vi "VIH Dialog - Project File List - Shortcut Menu Handler.vi"(6 "Menu Tag":string, 7 "Options":cluster{"Called from Master":bool}, 8 "Files":cluster{"Type":T1, "Path":path}[](array[cluster]), 10 "MenuRef":refnum<k9>, 11 "Event Type":T2) -> (3 "States spec":string)   [LabVIEW 2014]
doc: "::: VI Helpeks :::\nCopyright (c) 2000-2026 Konstantin Shifershteyn. All rights reserved."
uses:
  <vilib>/event_ctls.llb/lveventtype.ctl
  _VIH HelpGen - Palette.llb/VIH HelpGen Typedef - Palette - Item Type Enum.ctl
  _VIH Support Library.llb/VIH Utility - MENU - Create Menu (String).vi
panel:
  # "VI Helpeks\nCopyright (c) 2012-2026 Konstantin Shifershteyn"
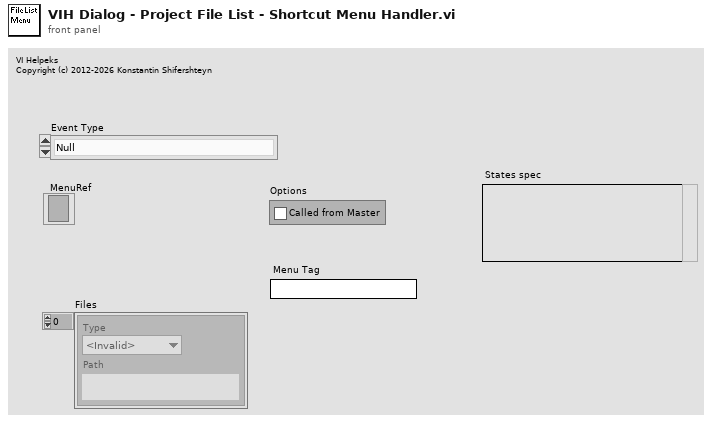
[diagram p1: front panel]
types:
  T1 = typedef "VIH HelpGen Typedef - Palette - Item Type Enum.ctl" = enum32{"<Invalid>", "<unknown>", "VI", "Menu", "LV Func", "Express VI", "Poly VI", "CTL", "HTML"}
  T2 = typedef "lveventtype.ctl" = enum32{"Null", "Timeout", "Annotation Menu Selection", "Annotation Menu Selection?", "App Instance Close", "App Instance Close?", "Autoscale Range Change", "Bookmark Info Change", "Cell Edit", "Cell Edit?", "Cursor Grab", "Cursor Grab?", "Cursor Menu Selection", "Cursor Menu Selection?", "Cursor Move", "Cursor Release", "Data Change", "Direction Change", "Display State Change", "Drag Ended", "Drag Enter", "Drag Leave", "Drag Over", "Drag Source Update", "Drag Starting", "Drag Starting?", "Drop", "Exec State Change", "Key Down", "Key Down?", "Key Repeat", "Key Repeat?", "Key Up", "Listbox Double Click", "Menu Activation?", "Menu Selection (App)", "Menu Selection? (App)", "Menu Selection (User)", "Mouse Down", "Mouse Down?", "Mouse Enter", "Mouse Leave", "Mouse Move", "Mouse Up", "Mouse Wheel", "NI Security User Change (App)", "Pane Size", "Panel Close", "Panel Close?", "Panel Resize", "Plot Attribute Change", "Scale Range Change", "Shortcut Menu Activation?", "Shortcut Menu Selection (App)", "Shortcut Menu Selection? (App)", "Shortcut Menu Selection (User)", "Tree Double Click", "Tree Drag", "Tree Drag?", "Tree Drop", "Tree Drop?", "Tree Item Close", "Tree Item Close?", "Tree Item Open", "Tree Item Open?", "User Event", "Value Change"}
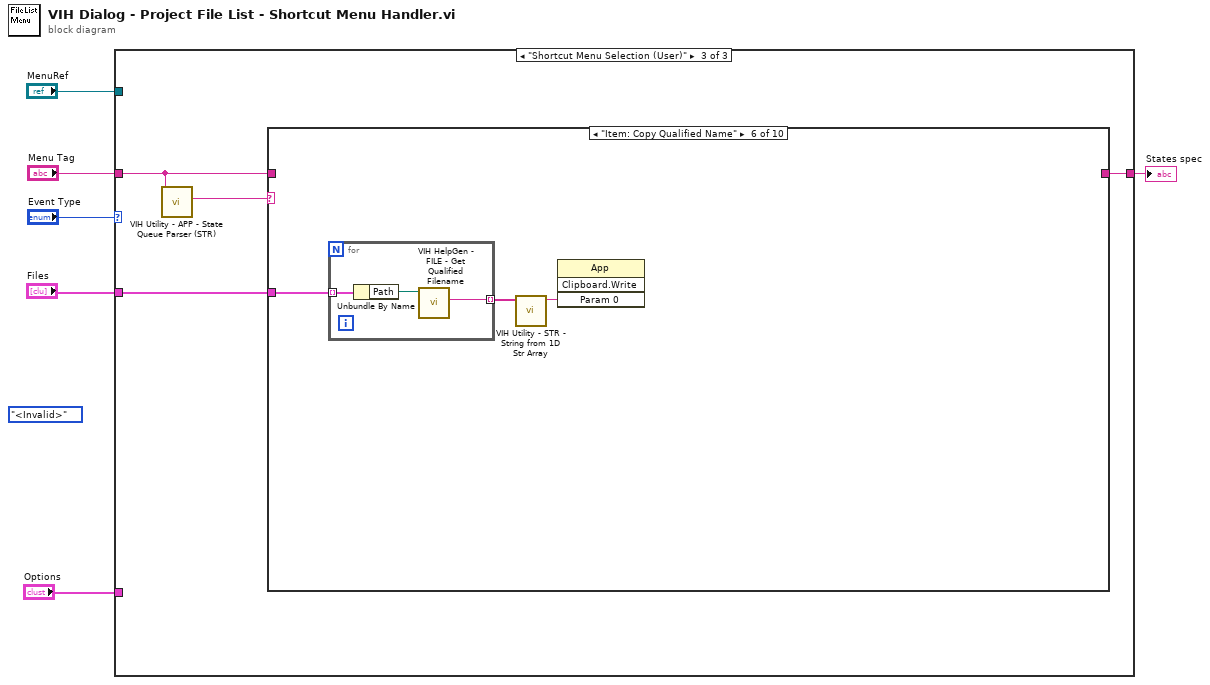
[diagram p0: block diagram]
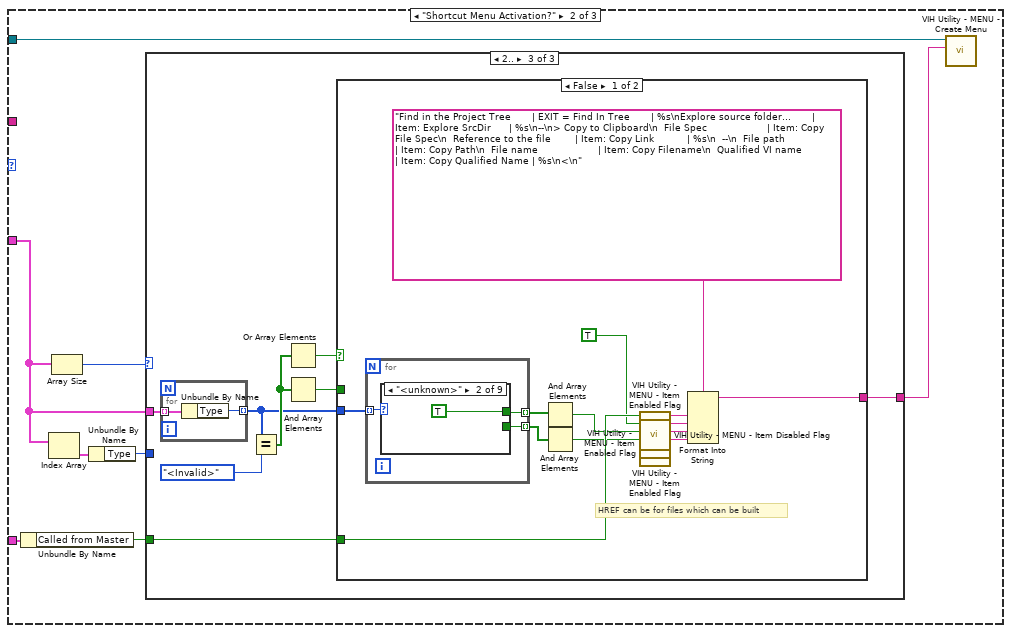
[diagram p3: hidden frame]
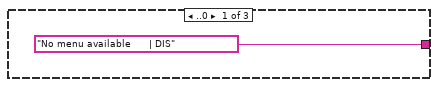
[diagram p4: hidden frame]
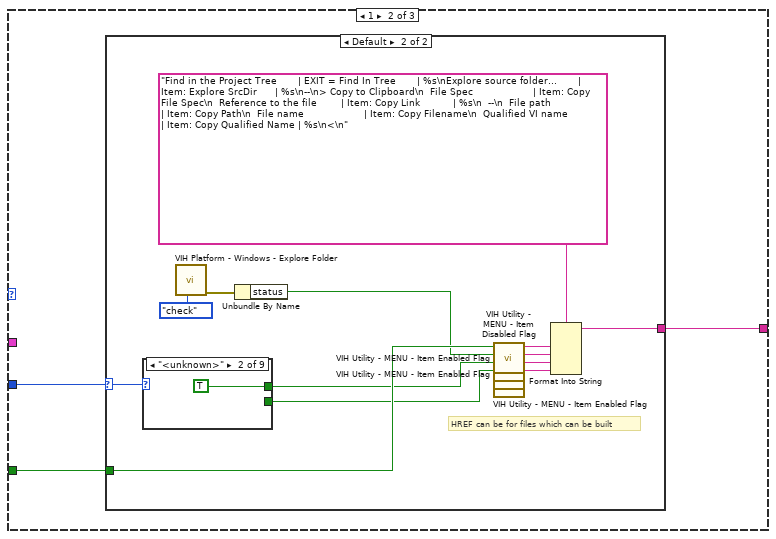
[diagram p5: hidden frame]
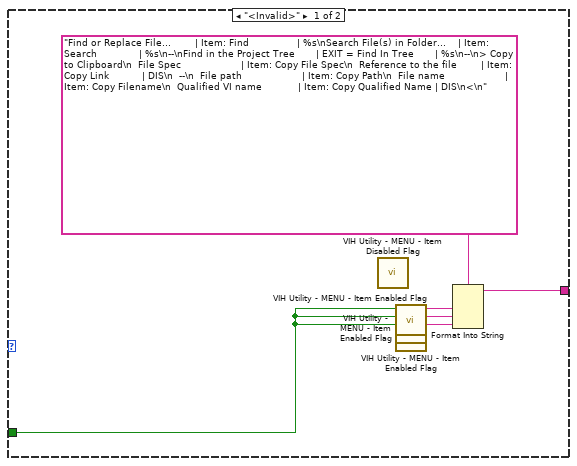
[diagram p6: hidden frame]
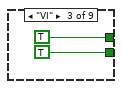
[diagram p8: hidden frame]
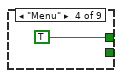
[diagram p9: hidden frame]
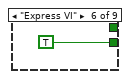
[diagram p11: hidden frame]
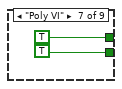
[diagram p12: hidden frame]
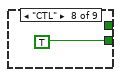
[diagram p13: hidden frame]
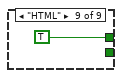
[diagram p14: hidden frame]
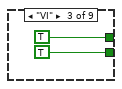
[diagram p16: hidden frame]
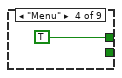
[diagram p17: hidden frame]
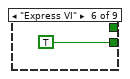
[diagram p19: hidden frame]
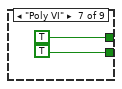
[diagram p20: hidden frame]
diagram:
  (unwired) VIH_HelpGen_Typedef_-_Palette_-_Item_Type_Enum."<Invalid>" ("Type")
  n1 = case shown="\"Shortcut Menu Selection (User)\"" "Event Type" {
    tunnel: "MenuRef" -> [_ w14 _]
    tunnel: [_ _ w92] -> w4
    tunnel: "Menu Tag" -> [_ _ w93]
    tunnel: "Files" -> [_ w7 w91]
    tunnel: "Options" -> [_ w12 _]
    frame Default {
    }
    frame "Shortcut Menu Activation?" {
      n2 = Unbundle By Name(w12) -> ("Called from Master"=w11:bool)
      n3 = Index Array(array=w7) -> (element=w9:cluster{"Type":T1, "Path":path})  [unwired: 1 in]
      n4 = Array Size(array=w7) -> (size(s)=w10:i32)
      n5 = Unbundle By Name(w9) -> ("Type"=w8:T1)
      n6 = case shown="2.." w10 {
        tunnel: ["No menu available      | DIS" w18 w54] -> w13
        tunnel: w11 -> [_ w17 w53]
        tunnel: w8 -> [_ w16 _]
        tunnel: w7 -> [_ _ w52]
        frame ..0 {
        }
        frame 1 {
          n7 = case shown="Default" w16 {
            selector: w16 -> [_ w33]
            tunnel: [w23 w36] -> w18
            tunnel: w17 -> [w19 w34]
            frame "<Invalid>" {
              n8 = call "VIH Utility - MENU - Item Disabled Flag.vi"() -> ()  [unwired: 11 in, 1 out]
              n9 = call "VIH Utility - MENU - Item Enabled Flag.vi"("Enable?"=w19) -> ("Disable flag"=w22:string)  [unwired: 10 in]
              n10 = call "VIH Utility - MENU - Item Enabled Flag.vi"("Enable?"=w19) -> ("Disable flag"=w21:string)  [unwired: 10 in]
              n11 = call "VIH Utility - MENU - Item Enabled Flag.vi"("Enable?"=w19) -> ("Disable flag"=w20:string)  [unwired: 10 in]
              n12 = Format Into String(format string="Find or Replace File...        | Item: Find                | %s\nSearch File(s) in Folder...    | Item: Search              | %s\n--\nFind in the Project Tree       | EXIT = Find In Tree       | %s\n--\n> Copy to Clipboard\n  File Spec                    | Item: Copy File Spec\n  Reference to the file        | Item: Copy Link           | DIS\n  --\n  File path                    | Item: Copy Path\n  File name                    | Item: Copy Filename\n  Qualified VI name            | Item: Copy Qualified Name | DIS\n<\n", w22, w21, w20) -> (resulting string=w23:string)  [unwired: 2 in, 1 out]
            }
            frame Default {
              # "HREF can be for files which can be built"
              n13 = case shown="\"<unknown>\"" w33 {
                tunnel: [_ TRUE TRUE TRUE _ _ TRUE _ TRUE] -> w27
                tunnel: [_ _ TRUE _ _ TRUE TRUE TRUE _] -> w26
                frame "<Invalid>" {
                }
                frame "<unknown>" {
                }
                frame "VI" {
                }
                frame "Menu" {
                }
                frame "LV Func" {
                }
                frame "Express VI" {
                }
                frame "Poly VI" {
                }
                frame "CTL" {
                }
                frame "HTML" {
                }
              }
              n14 = call "VIH Platform - Windows - Explore Folder.vi"("cmd (run)"=enum16{"run", "check"}."check") -> ("error out"=w30:errorcluster)  [unwired: 10 in]
              n15 = Unbundle By Name(w30) -> ("status"=w28:bool)
              n16 = call "VIH Utility - MENU - Item Enabled Flag.vi"("Enable?"=w34) -> ("Disable flag"=w35:string)  [unwired: 10 in]
              n17 = call "VIH Utility - MENU - Item Disabled Flag.vi"("Disable?"=w28) -> ("Disable flag"=w29:string)  [unwired: 10 in]
              n18 = call "VIH Utility - MENU - Item Enabled Flag.vi"("Enable?"=w27) -> ("Disable flag"=w32:string)  [unwired: 10 in]
              n19 = call "VIH Utility - MENU - Item Enabled Flag.vi"("Enable?"=w26) -> ("Disable flag"=w25:string)  [unwired: 10 in]
              n20 = Format Into String(format string="Find in the Project Tree       | EXIT = Find In Tree       | %s\nExplore source folder...       | Item: Explore SrcDir      | %s\n--\n> Copy to Clipboard\n  File Spec                    | Item: Copy File Spec\n  Reference to the file        | Item: Copy Link           | %s\n  --\n  File path                    | Item: Copy Path\n  File name                    | Item: Copy Filename\n  Qualified VI name            | Item: Copy Qualified Name | %s\n<\n", w35, w29, w32, w25) -> (resulting string=w36:string)  [unwired: 2 in, 1 out]
            }
          }
        }
        frame 2.. {
          n21 = for {
            tunnel: w52 -> [w90] mode=indexing
            tunnel: [w89] -> w47 mode=indexing
            n22 = Unbundle By Name(w90) -> ("Type"=w89:T1)
          }
          n23 = Equal?(x=w47, y=VIH_HelpGen_Typedef_-_Palette_-_Item_Type_Enum."<Invalid>" ("Type")) -> (x = y?=w50:bool[])
          n24 = Or Array Elements(Boolean array=w50) -> (logical OR=w49:bool)
          n25 = And Array Elements(Boolean array=w50) -> (logical AND=w48:bool)
          n26 = case shown="False" w49 {
            tunnel: [w66 w87] -> w54
            tunnel: w53 -> [w64 w81]
            tunnel: w48 -> [_ w80]
            tunnel: w47 -> [w60 _]
            frame False {
              # "HREF can be for files which can be built"
              n27 = for {
                tunnel: [w69] -> w62 mode=indexing
                tunnel: w60 -> [w70] mode=indexing
                tunnel: [w68] -> w57 mode=indexing
                n28 = case shown="\"<unknown>\"" w70 {
                  tunnel: [_ TRUE TRUE TRUE _ _ TRUE _ TRUE] -> w69
                  tunnel: [_ _ TRUE _ _ TRUE TRUE TRUE _] -> w68
                  frame "<Invalid>" {
                  }
                  frame "<unknown>" {
                  }
                  frame "VI" {
                  }
                  frame "Menu" {
                  }
                  frame "LV Func" {
                  }
                  frame "Express VI" {
                  }
                  frame "Poly VI" {
                  }
                  frame "CTL" {
                  }
                  frame "HTML" {
                  }
                }
              }
              n29 = And Array Elements(Boolean array=w62) -> (logical AND=w61:bool)
              n30 = And Array Elements(Boolean array=w57) -> (logical AND=w56:bool)
              n31 = call "VIH Utility - MENU - Item Enabled Flag.vi"("Enable?"=w64) -> ("Disable flag"=w65:string)  [unwired: 10 in]
              n32 = call "VIH Utility - MENU - Item Disabled Flag.vi"("Disable?"=TRUE) -> ("Disable flag"=w59:string)  [unwired: 10 in]
              n33 = call "VIH Utility - MENU - Item Enabled Flag.vi"("Enable?"=w61) -> ("Disable flag"=w63:string)  [unwired: 10 in]
              n34 = call "VIH Utility - MENU - Item Enabled Flag.vi"("Enable?"=w56) -> ("Disable flag"=w55:string)  [unwired: 10 in]
              n35 = Format Into String(format string="Find in the Project Tree       | EXIT = Find In Tree       | %s\nExplore source folder...       | Item: Explore SrcDir      | %s\n--\n> Copy to Clipboard\n  File Spec                    | Item: Copy File Spec\n  Reference to the file        | Item: Copy Link           | %s\n  --\n  File path                    | Item: Copy Path\n  File name                    | Item: Copy Filename\n  Qualified VI name            | Item: Copy Qualified Name | %s\n<\n", w65, w59, w63, w55) -> (resulting string=w66:string)  [unwired: 2 in, 1 out]
            }
            frame True {
              n36 = And(x=w80, y=w81) -> (x .and. y?=w82:bool)
              n37 = call "VIH Utility - MENU - Item Disabled Flag.vi"() -> ()  [unwired: 11 in, 1 out]
              n38 = call "VIH Utility - MENU - Item Enabled Flag.vi"("Enable?"=FALSE) -> ("Disable flag"=w84:string)  [unwired: 10 in]
              n39 = call "VIH Utility - MENU - Item Enabled Flag.vi"("Enable?"=w82) -> ("Disable flag"=w85:string)  [unwired: 10 in]
              n40 = call "VIH Utility - MENU - Item Enabled Flag.vi"("Enable?"=w81) -> ("Disable flag"=w88:string)  [unwired: 10 in]
              n41 = Format Into String(format string="Find or Replace File...        | Item: Find                | %s\nSearch File(s) in Folder...    | Item: Search              | %s\n--\nFind in the Project Tree       | EXIT = Find In Tree       | %s\n--\n> Copy to Clipboard\n  File Spec                    | Item: Copy File Spec\n  Reference to the file        | Item: Copy Link           | DIS\n  --\n  File path                    | Item: Copy Path\n  File name                    | Item: Copy Filename\n  Qualified VI name            | Item: Copy Qualified Name | DIS\n<\n", w84, w85, w88) -> (resulting string=w87:string)  [unwired: 2 in, 1 out]
            }
          }
        }
      }
      n42 = call-poly "VIH Utility - MENU - Create Menu.vi"("Menu Description"=w13, "menu"=w14) -> ()  [unwired: 8 in, 2 out]
    }
    frame "Shortcut Menu Selection (User)" {
      n43 = call "VIH Utility - APP - State Queue Parser (STR).vi"("input queue"=w93) -> ("state"=w94:string)  [unwired: 5 in, 3 out]
      n44 = case shown="\"Item: Copy Qualified Name\"" w94 {
        tunnel: [w95 _ _ _ _ _ _ w133 w142 _] -> w92
        tunnel: w93 -> [w96 _ _ _ _ _ _ _ _ _]
        tunnel: w91 -> [_ w103 w109 w116 w121 w127 _ w137 w141 w151]
        frame Default {
          n45 = Match Pattern(string=w96, regular expression=";$") -> (offset past match=w97:i32)  [unwired: 1 in, 3 out]
          n46 = case shown="..-1" w97 {
            tunnel: w96 -> [w101 w102]
            tunnel: [w100 w102] -> w95
            frame ..-1 {
              n47 = Concatenate Strings(w101, ";" ("string")) -> (w100:string)
            }
            frame 0.. {
            }
          }
        }
        frame "Item: Copy File Spec" {
          n48 = for {
            tunnel: [w108] -> w105 mode=indexing
            tunnel: w103 -> [w107] mode=indexing
            n49 = Unbundle By Name(w107) -> ("Path"=w108:path)
          }
          n50 = call "VIH XML - File Array to-from XML String.vi"("cmd (check)"=enum16{"check", "parse", "format"}."format", "Files in"=w105) -> ("XML out"=w106:string)  [unwired: 6 in, 3 out]
          n51 = invoke class="App" method="Clipboard.Write"("Param 0"=w106) -> ()  [unwired: 3 in, 4 out]
        }
        frame "Item: Copy Link" {
          n52 = for {
            tunnel: [w114] -> w111 mode=indexing
            tunnel: w109 -> [w113] mode=indexing
            n53 = Unbundle By Name(w113) -> ("Path"=w112:path)
            n54 = call "VIH HelpGen - HREF - Build.vi"("File Path"=w112) -> ("A HREF"=w114:string)  [unwired: 10 in]
          }
          n55 = call "VIH Utility - STR - String from 1D Str Array.vi"("Array in"=w111) -> ("String out"=w110:string)  [unwired: 6 in]
          n56 = invoke class="App" method="Clipboard.Write"("Param 0"=w110) -> ()  [unwired: 3 in, 4 out]
        }
        frame "Item: Copy Path" {
          n57 = for {
            tunnel: w116 -> [w120] mode=indexing
            tunnel: [w119] -> w115 mode=indexing
            n58 = Unbundle By Name(w120) -> ("Path"=w118:path)
            n59 = Path To String(path=w118) -> (string=w119:string)
          }
          n60 = call "VIH Utility - STR - String from 1D Str Array.vi"("Array in"=w115) -> ("String out"=w117:string)  [unwired: 6 in]
          n61 = invoke class="App" method="Clipboard.Write"("Param 0"=w117) -> ()  [unwired: 3 in, 4 out]
        }
        frame "Item: Copy Filename" {
          n62 = for {
            tunnel: [w126] -> w123 mode=indexing
            tunnel: w121 -> [w125] mode=indexing
            n63 = Unbundle By Name(w125) -> ("Path"=w124:path)
            n64 = Strip Path(path=w124) -> (name=w126:string)  [unwired: 1 out]
          }
          n65 = call "VIH Utility - STR - String from 1D Str Array.vi"("Array in"=w123) -> ("String out"=w122:string)  [unwired: 6 in]
          n66 = invoke class="App" method="Clipboard.Write"("Param 0"=w122) -> ()  [unwired: 3 in, 4 out]
        }
        frame "Item: Copy Qualified Name" {
          n67 = for {
            tunnel: [w130] -> w129 mode=indexing
            tunnel: w127 -> [w132] mode=indexing
            n68 = Unbundle By Name(w132) -> ("Path"=w131:path)
            n69 = call "VIH HelpGen - FILE - Get Qualified Filename.vi"("File Path"=w131) -> ("Qualified name"=w130:string)  [unwired: 9 in, 1 out]
          }
          n70 = call "VIH Utility - STR - String from 1D Str Array.vi"("Array in"=w129) -> ("String out"=w128:string)  [unwired: 6 in]
          n71 = invoke class="App" method="Clipboard.Write"("Param 0"=w128) -> ()  [unwired: 3 in, 4 out]
        }
        frame "------------------------------ 1" {
        }
        frame "Item: Find" {
          n72 = Index Array(array=w137) -> (element=w136:cluster{"Type":T1, "Path":path})  [unwired: 1 in]
          n73 = Unbundle By Name(w136) -> ("Path"=w135:path)
          n74 = Format Into String(format string="Find File = %s;", w135) -> (resulting string=w133:string)  [unwired: 2 in, 1 out]
        }
        frame "Item: Search" {
          n75 = for {
            tunnel: w141 -> [w146] mode=indexing
            tunnel: [w144] -> w140 mode=indexing
            n76 = Unbundle By Name(w146) -> ("Path"=w145:path)
            n77 = Path To String(path=w145) -> (string=w144:string)
          }
          n78 = call "VIH Utility - STR - String from 1D Str Array.vi"("delimiter ('\\n')"="?" ("delimiter ('\\n')"), "Array in"=w140) -> ("String out"=w139:string)  [unwired: 5 in]
          n79 = Format Into String(format string="Search Files = %s;", w139) -> (resulting string=w142:string)  [unwired: 2 in, 1 out]
        }
        frame "Item: Explore SrcDir" {
          n80 = Index Array(array=w151) -> (element=w150:cluster{"Type":T1, "Path":path})  [unwired: 1 in]
          n81 = Unbundle By Name(w150) -> ("Path"=w147:path)
          n82 = call "VIH Platform - Windows - Explore Folder.vi"("cmd (run)"=enum16{"run", "check"}."run", "exe/doc/dir path"=w147) -> ("error out"=w148:errorcluster)  [unwired: 9 in]
          n83 = call <vilib>:"Simple Error Handler.vi"("error in (no error)"=w148) -> ()  [unwired: 4 in, 5 out]
        }
      }
    }
  }
  "States spec" <- w4
